vi "measure CE OOB Trigger Level.vi"(8 "error in (no error)":errorcluster, 11 "SA Measurement in":refnum<class "SA Measurement.lvclass">) -> (0 "error out":errorcluster, 3 "SA Measurement out":refnum<class "SA Measurement.lvclass">)   [LabVIEW 2023, in "Spectrum Analyzer.lvlib" / "SA Measurement.lvclass"]
uses:
  SA Measurement.lvclass
  SA Measurement.lvclass/SA Measurement.ctl
  TYPE DEFINITION/TYPE RBW and VBW Select.ctl
  Spectrum Analyzer.lvlib
  TYPE DEFINITION/TYPE Marker Peak Search Type.ctl
  Interface_Spectrum/Interface_Spectrum.lvclass
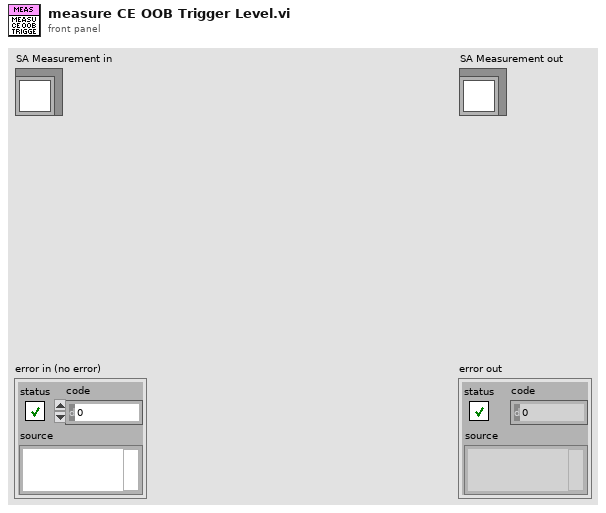
[diagram p1: front panel]
types:
  T1 = typedef "Spectrum Analyzer.lvlib/TYPE Marker Peak Search Type.ctl" = enum16{"Max", "Next Peak"}
  T2 = typedef "Spectrum Analyzer.lvlib/TYPE RBW and VBW Select.ctl" = enum16{"Res BW", "Video BW"}
  T3 = typedef "Spectrum Analyzer.lvlib/TYPE Y-axis Unit.ctl" = enum16{"dBm", "dBmV", "dBuV", "dBpW", "Volt", "Ampere", "Watt"}
  T4 = typedef "Spectrum Analyzer.lvlib/TYPE Display Trace Mode Select.ctl" = enum16{"Clear Write", "Max Hold", "Min Hold", "Average", "View"}
  T5 = typedef "Spectrum Analyzer.lvlib/TYPE Detect Mode Select.ctl" = enum16{"Det Auto (Normal)", "Auto Peak", "Positive Peak", "Negative Peak", "Sample", "RMS", "Average", "Quasipeak", "CISPR Average", "RMS Average"}
  T6 = cluster{"Trace Mode":T4, "Detector Type":T5, "Detect Auto?":bool}[]
  T7 = typedef "Spectrum Analyzer.lvlib/TYPE Marker Value.ctl" = cluster{"X-axis":dbl, "Y-axis":dbl}
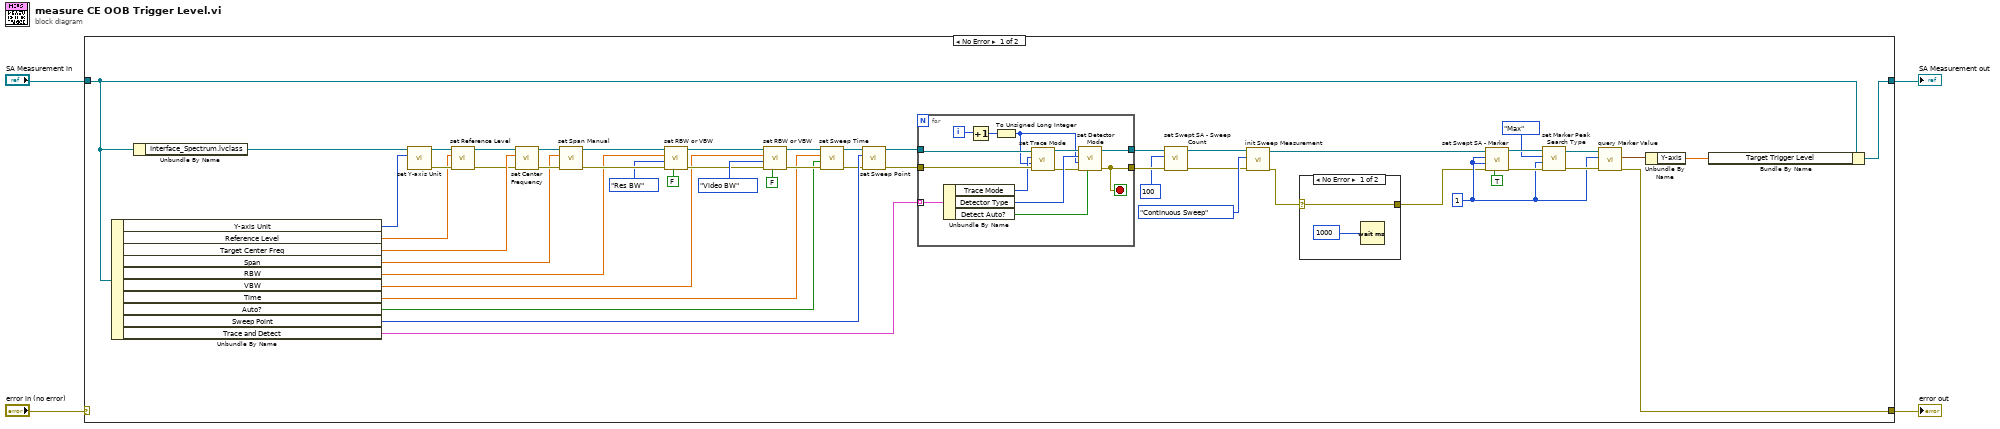
[diagram p0: block diagram]
diagram:
  n1 = case shown="No Error" "error in (no error)" {
    selector: "error in (no error)" -> [_ w74]
    tunnel: [w27 w74] -> w1
    tunnel: [w11 w73] -> w3
    tunnel: "SA Measurement in" -> [w13 w73]
    frame No Error {
      w28 = 1 ("Index")
      n2 = Unbundle By Name(w13) -> ("Y-axis Unit"=w42:T3, "Reference Level"=w24:dbl, "Target Center Freq"=w56:dbl, "Span"=w53:dbl, "RBW"=w50:dbl, "VBW"=w43:dbl, "Time"=w39:dbl, "Auto?"=w38:bool, "Sweep Point"=w21:u32, "Trace and Detect"=w37:T6)
      n3 = Unbundle By Name(w13) -> ("Interface_Spectrum.lvclass"=w10:refnum<class "Interface_Spectrum.lvclass">)
      n4 = call-dynamic "set Y-axis Unit.vi"("Y-axis Unit"=w42, "Interface_Spectrum in"=w10) -> ("error out"=w25:errorcluster, "Interface_Spectrum out"=w26:refnum<class "Interface_Spectrum.lvclass">)  [unwired: 8 in]
      n5 = call-dynamic "set Reference Level.vi"("error in (no error)"=w25, "Reference Level"=w24, "Interface_Spectrum in"=w26) -> ("error out"=w22:errorcluster, "Interface_Spectrum out"=w23:refnum<class "Interface_Spectrum.lvclass">)  [unwired: 7 in]
      n6 = call-dynamic "set Center Frequency.vi"("error in (no error)"=w22, "Center Frequency (Hz)"=w56, "Interface_Spectrum in"=w23) -> ("error out"=w54:errorcluster, "Interface_Spectrum out"=w55:refnum<class "Interface_Spectrum.lvclass">)  [unwired: 7 in]
      n7 = call-dynamic "set Span Manual.vi"("error in (no error)"=w54, "Span (Hz)"=w53, "Interface_Spectrum in"=w55) -> ("error out"=w51:errorcluster, "Interface_Spectrum out"=w52:refnum<class "Interface_Spectrum.lvclass">)  [unwired: 7 in]
      n8 = call-dynamic "set RBW or VBW.vi"("BW Auto?"=FALSE, "error in (no error)"=w51, "BW Type"=TYPE_RBW_and_VBW_Select."Res BW", "BW Value (Hz)"=w50, "Interface_Spectrum in"=w52) -> ("error out"=w44:errorcluster, "Interface_Spectrum out"=w45:refnum<class "Interface_Spectrum.lvclass">)  [unwired: 5 in]
      n9 = call-dynamic "set RBW or VBW.vi"("BW Auto?"=FALSE, "error in (no error)"=w44, "BW Type"=TYPE_RBW_and_VBW_Select."Video BW", "BW Value (Hz)"=w43, "Interface_Spectrum in"=w45) -> ("error out"=w40:errorcluster, "Interface_Spectrum out"=w41:refnum<class "Interface_Spectrum.lvclass">)  [unwired: 5 in]
      n10 = call-dynamic "set Sweep Time.vi"("error in (no error)"=w40, "Sweep Time Auto?"=w38, "Sweep Time(sec)"=w39, "Interface_Spectrum in"=w41) -> ("error out"=w19:errorcluster, "Interface_Spectrum out"=w20:refnum<class "Interface_Spectrum.lvclass">)  [unwired: 6 in]
      n11 = call-dynamic "set Sweep Point.vi"("error in (no error)"=w19, "Sweep Point"=w21, "Interface_Spectrum in"=w20) -> ("error out"=w17:errorcluster, "Interface_Spectrum out"=w18:refnum<class "Interface_Spectrum.lvclass">)  [unwired: 7 in]
      n12 = for {
        tunnel: w18 -> [w71]
        tunnel: w17 -> [w70]
        tunnel: w37 -> [w72] mode=indexing
        tunnel: [w60] -> w35
        tunnel: [w61] -> w36
        i -> [w69]
        stop <- w60 stop-if-true
        n13 = Unbundle By Name(w72) -> ("Trace Mode"=w67:T4, "Detector Type"=w65:T5, "Detect Auto?"=w62:bool)
        n14 = Increment(x=w69) -> (x+1=w68:i32)
        n15 = To Unsigned Long Integer(number=w68) -> (unsigned 32bit integer=w63:u32)
        n16 = call-dynamic "set Trace Mode.vi"("error in (no error)"=w70, "Trace Index"=w63, "Trace Mode"=w67, "Interface_Spectrum in"=w71) -> ("error out"=w64:errorcluster, "Interface_Spectrum out"=w66:refnum<class "Interface_Spectrum.lvclass">)  [unwired: 6 in]
        n17 = call-dynamic "set Detector Mode.vi"("Detect Auto?"=w62, "error in (no error)"=w64, "Trace Index"=w63, "Detector Type"=w65, "Interface_Spectrum in"=w66) -> ("error out"=w60:errorcluster, "Interface_Spectrum out"=w61:refnum<class "Interface_Spectrum.lvclass">)  [unwired: 5 in]
      }
      n18 = call-dynamic "set Swept SA - Sweep Count.vi"("error in (no error)"=w35, "Sweep Count"=u32 100, "Interface_Spectrum in"=w36) -> ("error out"=w6:errorcluster, "Interface_Spectrum out"=w8:refnum<class "Interface_Spectrum.lvclass">)  [unwired: 7 in]
      n19 = call-dynamic "init Sweep Measurement.vi"("error in (no error)"=w6, "Sweep Measurement Mode"=enum16{"Single Sweep", "Continuous Sweep"}."Continuous Sweep", "Interface_Spectrum in"=w8) -> ("error out"=w7:errorcluster, "Interface_Spectrum out"=w5:refnum<class "Interface_Spectrum.lvclass">)  [unwired: 7 in]
      n20 = case shown="No Error" w7 {
        selector: w7 -> [w57 w59]
        tunnel: [w57 w59] -> w15
        frame No Error {
          n21 = Wait (ms)(milliseconds to wait=u32 1000) -> ()  [unwired: 1 out]
        }
        frame Error {
        }
      }
      n22 = call-dynamic "set Swept SA - Marker.vi"("On?"=TRUE, "error in (no error)"=w15, "trace"=w28, "Index"=w28, "Interface_Spectrum in"=w5) -> ("error out"=w32:errorcluster, "Interface_Spectrum out"=w33:refnum<class "Interface_Spectrum.lvclass">)  [unwired: 5 in]
      n23 = call-dynamic "set Marker Peak Search Type.vi"("error in (no error)"=w32, "Marker Index"=w28, "Peak Search Type"=TYPE_Marker_Peak_Search_Type."Max", "Interface_Spectrum in"=w33) -> ("error out"=w29:errorcluster, "Interface_Spectrum out"=w30:refnum<class "Interface_Spectrum.lvclass">)  [unwired: 6 in]
      n24 = call-dynamic "query Marker Value.vi"("error in (no error)"=w29, "Marker Index"=w28, "Interface_Spectrum in"=w30) -> ("error out"=w27:errorcluster, "Marker Value"=w14:T7)  [unwired: 6 in, 1 out]
      n25 = Unbundle By Name(w14) -> ("Y-axis"=w12:dbl)
      n26 = Bundle By Name(cluster=w13, "Target Trigger Level"=w12) -> (w11:refnum<class "SA Measurement.lvclass">)
    }
    frame Error {
    }
  }
  "error out" <- w1
  "SA Measurement out" <- w3
